vi "Create Indicator.vi"(0 "result cluster":refnum<vi>, 5 "vi reference":refnum<vi>, 7 "ctl refnum":refnum<vi>, 11 "error in":errorcluster) -> (15 "error out":errorcluster)   [LabVIEW 2021, in "Converter.lvlib"]
uses:
  Converter.lvlib
  <vilib>/Utility/miscctls.llb/LVPositionTypeDef.ctl
  <vilib>/numeric/LVNumericRepresentation.ctl
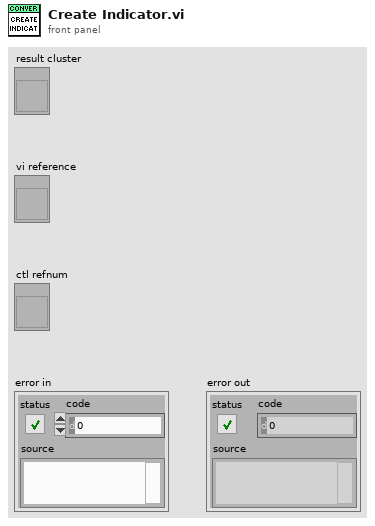
[diagram p1: front panel]
types:
  T1 = typedef "LVPositionTypeDef.ctl" = cluster{"Left":i32, "Top":i32}
  T2 = typedef "LVNumericRepresentation.ctl" = enum32{"Extended Precision", "Double Precision", "Single Precision", "Long", "Word", "Byte", "Unsigned Long", "Unsigned Word", "Unsigned Byte", "Complex Extended", "Complex Double", "Complex Single", "Quad", "Unsigned Quad", "Fixed-Point"}
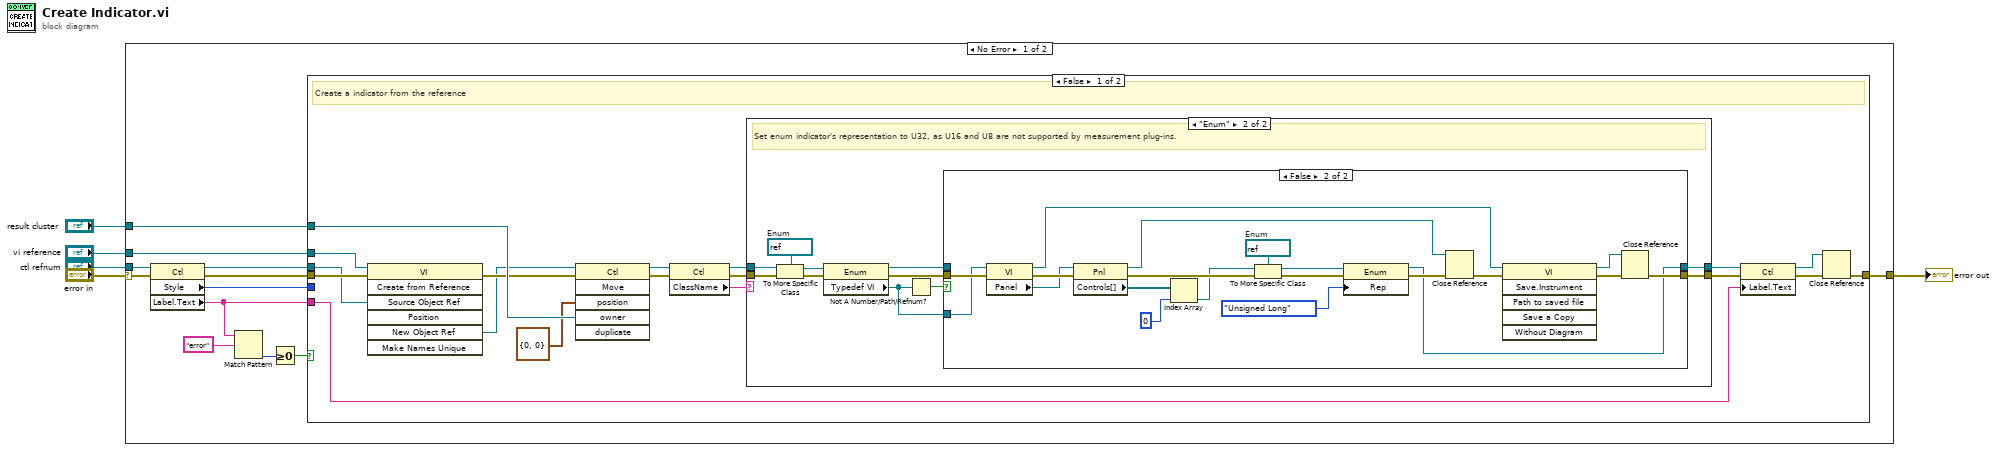
[diagram p0: block diagram]
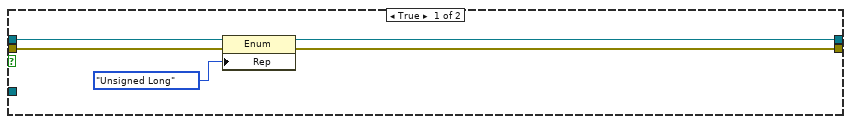
[diagram p3: hidden frame]
diagram:
  n1 = case shown="No Error" "error in" {
    selector: "error in" -> [w17 w75]
    tunnel: "ctl refnum" -> [w16 _]
    tunnel: "vi reference" -> [w14 _]
    tunnel: [w10 w75] -> w2
    tunnel: "result cluster" -> [w8 _]
    frame No Error {
      n2 = property class="Ctl"(reference=w16, error in=w17) -> (reference out=w15:refnum<vi>, error out=w9:errorcluster, "Style"=w7:u32, "Label.Text"=w11:string)
      n3 = Match Pattern(string=w11, regular expression="error") -> (offset past match=w6:i32)  [unwired: 1 in, 3 out]
      n4 = Greater Or Equal To 0?(x=w6) -> (x >= 0?=w13:bool)
      n5 = case shown="False" w13 {
        tunnel: w7 -> [_ _]
        tunnel: w8 -> [w33 _]
        tunnel: w9 -> [w35 w74]
        tunnel: w15 -> [w32 _]
        tunnel: [w34 w74] -> w10
        tunnel: w11 -> [w24 _]
        tunnel: w14 -> [w31 _]
        frame False {
          # "Create a indicator from the reference"
          n6 = invoke class="VI" method="Create from Reference"(reference=w31, error in=w35, "Source Object Ref"=w32) -> (error out=w30:errorcluster, "New Object Ref"=w29:refnum<vi>)  [unwired: 4 in, 5 out]
          n7 = invoke class="Ctl" method="Move"(reference=w29, error in=w30, "position"=T1 {"Left"=0, "Top"=0}, "owner"=w33) -> (reference out=w23:refnum<vi>, error out=w25:errorcluster)  [unwired: 2 in, 4 out]
          n8 = property class="Ctl"(reference=w23, error in=w25) -> (reference out=w21:refnum<vi>, error out=w22:errorcluster, "ClassName"=w18:string)
          n9 = case shown="\"Enum\"" w18 {
            tunnel: [w37 w43] -> w19
            tunnel: w22 -> [w37 w48]
            tunnel: w21 -> [w36 w47]
            tunnel: [w36 w42] -> w20
            frame Default {
            }
            frame "Enum" {
              w46 = refnum<vi> refnum  # Enum
              # "Set enum indicator's representation to U32, as U16 and U8 are not supported by measurement plug-ins."
              n10 = To More Specific Class(target class=w46, reference=w47, error in=w48) -> (specific class reference=w41:refnum<vi>, error out=w40:errorcluster)
              n11 = property class="Enum"(reference=w41, error in=w40) -> (reference out=w44:refnum<vi>, error out=w45:errorcluster, "Typedef VI"=w38:refnum<vi>)
              n12 = Not A Number/Path/Refnum?(number/path/refnum=w38) -> (NaN/Path/Refnum?=w39:bool)
              n13 = case shown="False" w39 {
                tunnel: w45 -> [w53 w73]
                tunnel: w44 -> [w51 _]
                tunnel: [w52 w56] -> w43
                tunnel: [w50 w54] -> w42
                tunnel: w38 -> [_ w71]
                frame True {
                  n14 = property class="Enum"(reference=w51, error in=w53, "Rep"=LVNumericRepresentation."Unsigned Long" ("Representation")) -> (reference out=w50:refnum<vi>, error out=w52:errorcluster)
                }
                frame False {
                  w64 = refnum<vi> refnum  # Enum
                  n15 = property class="VI"(reference=w71, error in=w73) -> (reference out=w57:refnum<vi>, error out=w72:errorcluster, "Panel"=w69:refnum<vi>)
                  n16 = property class="Pnl"(reference=w69, error in=w72) -> (reference out=w59:refnum<vi>, error out=w70:errorcluster, "Controls[]"=w61:refnum<vi>[])
                  n17 = Index Array(array=w61, index=0) -> (element=w66:refnum<vi>)
                  n18 = To More Specific Class(target class=w64, reference=w66, error in=w70) -> (specific class reference=w65:refnum<vi>, error out=w67:errorcluster)
                  n19 = property class="Enum"(reference=w65, error in=w67, "Rep"=LVNumericRepresentation."Unsigned Long" ("Representation")) -> (reference out=w54:refnum<vi>, error out=w62:errorcluster)
                  n20 = Close Reference(reference=w59, error in (no error)=w62) -> (error out=w60:errorcluster)
                  n21 = invoke class="VI" method="Save.Instrument"(reference=w57, error in=w60) -> (reference out=w55:refnum<vi>, error out=w58:errorcluster)  [unwired: 4 in, 4 out]
                  n22 = Close Reference(reference=w55, error in (no error)=w58) -> (error out=w56:errorcluster)
                }
              }
            }
          }
          n23 = property class="Ctl"(reference=w20, error in=w19, "Label.Text"=w24) -> (reference out=w26:refnum<vi>, error out=w27:errorcluster)
          n24 = Close Reference(reference=w26, error in (no error)=w27) -> (error out=w34:errorcluster)
        }
        frame True {
          # "Ignore it is error indicator"
        }
      }
    }
    frame Error {
    }
  }
  "error out" <- w2
